vi "read_calibration_config.vi"(8 "error in":errorcluster, 11 "Config file path":path=path "C:/Users/TDT/Box/Electrical Nerve Block Institute/Software/LabVIEW/tSNIP/calibration_config.csv") -> (0 "error out":errorcluster, 2 "Num Points":i32, 3 "Config Parameters":dbl[][](array[numeric]))   [LabVIEW 2025, in "tSNIP.lvlib"]
uses:
  tSNIP.lvlib
  <vilib>/Utility/file.llb/Read Delimited Spreadsheet (DBL).vi
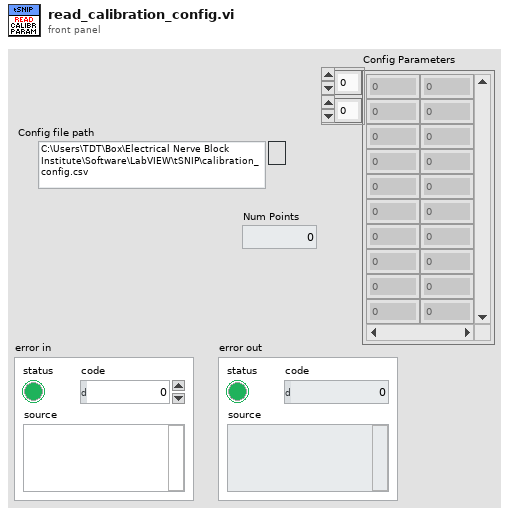
[diagram p1: front panel]
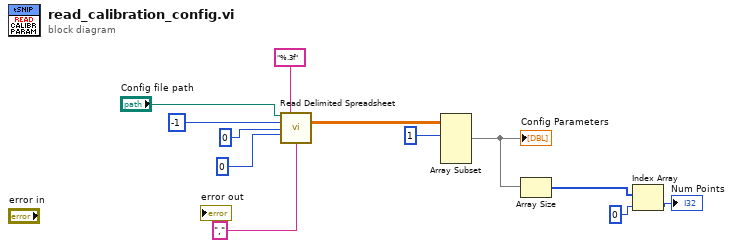
[diagram p0: block diagram]
diagram:
  n1 = call-poly <vilib>:"Read Delimited Spreadsheet.vi"("file path (dialog if empty)"="Config file path", "format (%.3f)"="%.3f", "number of rows (all:-1)"=-1, "start of read offset (chars.:0)"=0, "max characters/row  (no limit:0)"=0, "delimiter (\\t)"="," ("delimiter (\\t)")) -> ("all rows"=w6:dbl[][])  [unwired: 4 in, 5 out]
  n2 = Array Subset(array=w6, index (row)=1 ("index")) -> (w4:dbl[][])  [unwired: 3 in]
  "Config Parameters" <- w4
  n3 = Array Size(array=w4) -> (size(s)=w2:i32[])
  n4 = Index Array(array=w2, index=0) -> (element=→"Num Points":i32)
